vi "add_sub_vi.vi"(8 "error in (no error)":errorcluster, 9 "SubVI":refnum<class "HierarchyNode.lvclass">, 10 "VI":refnum<class "HierarchyNode.lvclass">, 11 "VIHierarchyGraph in":refnum<class "HierarchyGraph.lvclass">) -> (0 "error out":errorcluster, 1 "edge unchanged?":bool, 2 "edge already included?":bool, 3 "VIHierarchyGraph out":refnum<class "HierarchyGraph.lvclass">)   [LabVIEW 2020, in "vi-hierarchy.lvlib" / "HierarchyGraph.lvclass"]
uses:
  HierarchyGraph.lvclass
  VINode/HierarchyNode.lvclass
  home/jki/Projects/gaia/src/dragon-desktop/source/submodules/graph-api-labview/source/api/Node/Node.lvclass
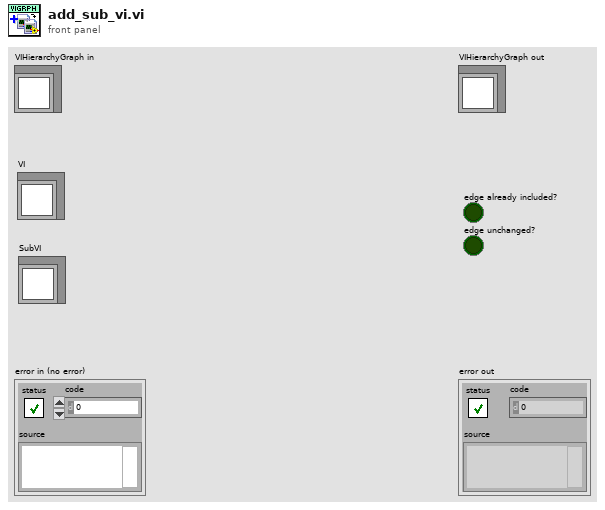
[diagram p1: front panel]
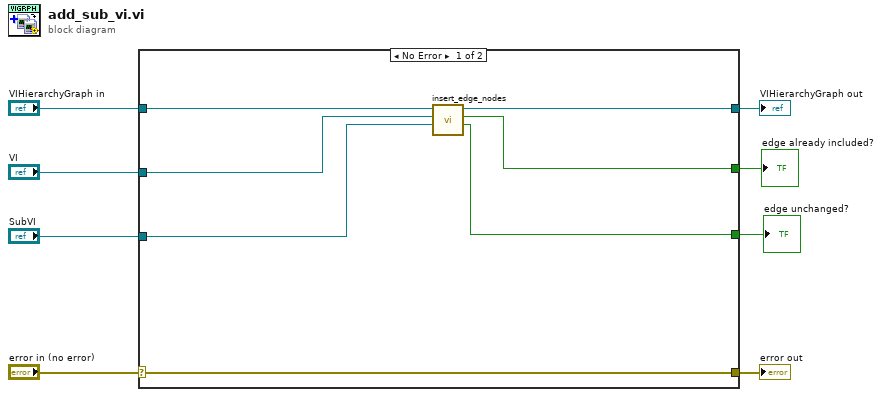
[diagram p0: block diagram]
diagram:
  n1 = case shown="No Error" "error in (no error)" {
    selector: "error in (no error)" -> [w15 w17]
    tunnel: [w15 w17] -> w7
    tunnel: [w13 w16] -> w5
    tunnel: "VIHierarchyGraph in" -> [w14 w16]
    tunnel: "VI" -> [w12 _]
    tunnel: "SubVI" -> [w11 _]
    tunnel: [w10 _] -> w2
    tunnel: [w9 _] -> w1
    frame No Error {
      n2 = call-dynamic "insert_edge_nodes.vi"("node-b"=w11, "node-a"=w12, "graph"=w14) -> ("edge unchanged?"=w9:bool, "edge already included?"=w10:bool, "graph out"=w13:refnum<class "HierarchyGraph.lvclass">)  [unwired: 5 in, 1 out]
    }
    frame Error {
    }
  }
  "error out" <- w7
  "VIHierarchyGraph out" <- w5
  "edge already included?" <- w2
  "edge unchanged?" <- w1
